vi "Test_tempo_realtime.vi"() -> ()   [LabVIEW 2017]
uses:
  <vilib>/Platform/TimedLoop/XDataNode/XDataNode.xnode
  <vilib>/Platform/TimedLoop/XDataNode/nitl_modes.ctl
  <vilib>/Platform/TimedLoop/XDataNode/XDNodeRunTimeDep.lvlib
  <vilib>/Platform/TimedLoop/XDataNode/wakeup.ctl
  <vilib>/Platform/TimedLoop/XDataNode/timing_clust.ctl
panel:
  out "Timer":u32 caption="Tick Count(mSec)"
  out "Tempo":bool
  in  "Timer":u32
  in  "Tempo":bool
  out "VI END":bool=TRUE
  out "Etat VI":enum16{""}(ring)
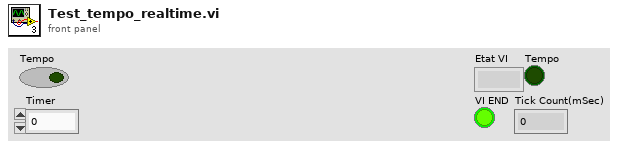
[diagram p1: front panel]
types:
  T1 = typedef "XDNodeRunTimeDep.lvlib/timing_clust.ctl" = cluster{"Expected End [f-1]":u64, "Actual End [f-1]":u64, "Finished Late? [f-1]":bool, "Expected End [i-1]":u64, "Actual End [i-1]":u64, "Finished Late? [i-1]":bool, "Expected Start [i]":u64, "Actual Start [i]":u64, "Expected Start [f]":u64, "Actual Start [f]":u64, "Source Name":string, "Structure Name":string, "Period":i64, "Deadline":i64, "Offset":i64, "Start":i64, "Priority":i32, "Timeout":i32, "Mode":T2, "Wakeup Reason":T3, "Error":errorcluster, "Source Type":string, "Secondary Source Type":string, "Global End Time":u64, "Global Start Time":u64, "Frame Duration":u64, "Iteration Duration":u64, "Assigned CPU":i32, "I/O Scan Engine Mode":u32}
  T2 = typedef "XDNodeRunTimeDep.lvlib/nitl_modes.ctl" = enum32{"No Change", "Process missed periods, maintain original phase", "Discard missed periods, maintain original phase", "Process missed periods, ignore original phase", "Discard missed periods, ignore original phase"}
  T3 = typedef "XDNodeRunTimeDep.lvlib/wakeup.ctl" = enum32{"Normal", "Aborted", "Asynchronous wakeup", "Timing source error", "Timed loop error", "Timeout"}
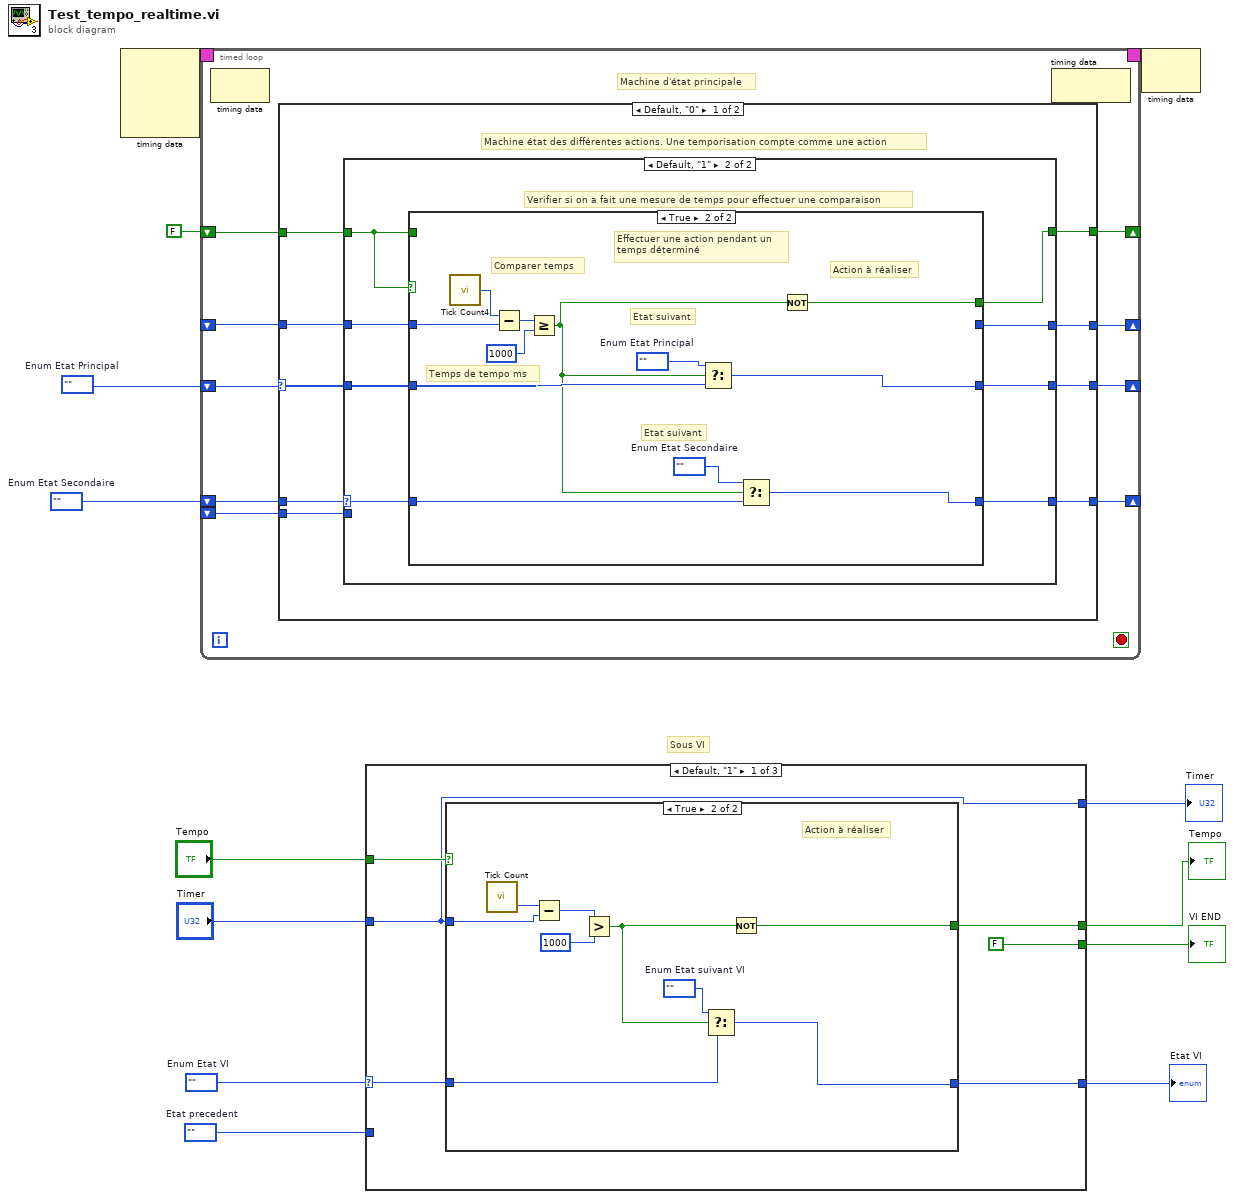
[diagram p0: block diagram]
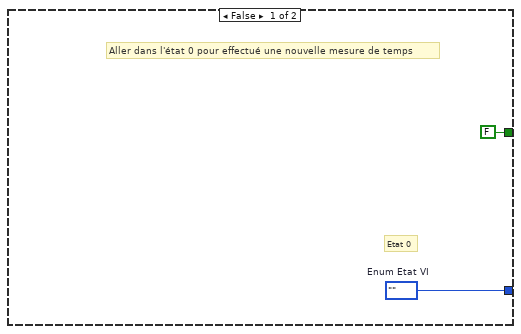
[diagram p2: hidden frame]
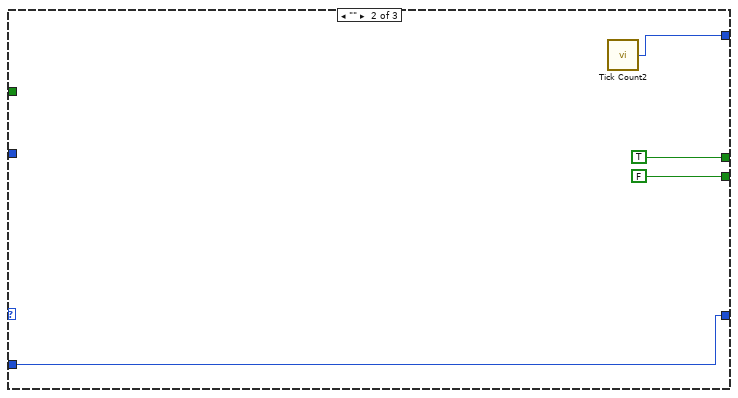
[diagram p3: hidden frame]
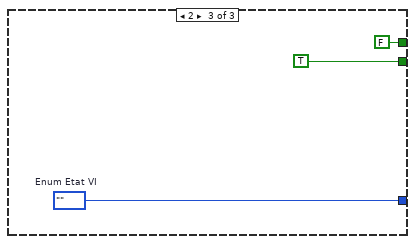
[diagram p4: hidden frame]
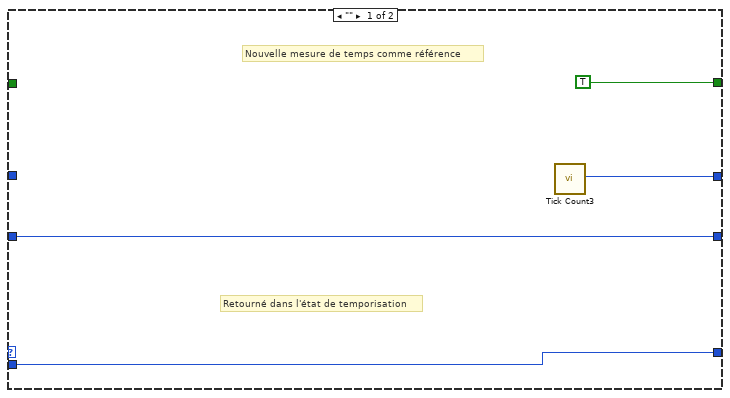
[diagram p5: hidden frame]
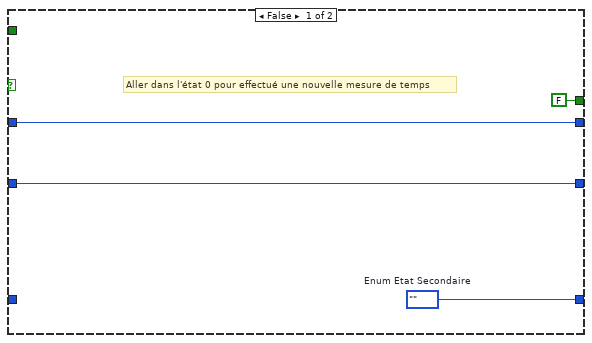
[diagram p6: hidden frame]
diagram:
  w2 = enum16{""}.""  # Etat precedent
  w1 = enum16{""}.""  # Enum Etat VI
  w10 = enum16{""}.""  # Enum Etat Secondaire
  w11 = enum16{""}.""  # Enum Etat Principal
  # "Sous VI"
  n1 = node-c288() -> (w13:T1)  [unwired: 4 in]
  n2 = timed-loop {
    timing: w13 -> [_]
    timing-out: [_] -> w12
    shift-right: [w16] -> _
    shift-left: w11 -> [w22]
    shift-right: [w18] -> _
    shift-left: w10 -> [w21]
    shift-right: [w20] -> _
    shift-left: _ -> [w19]
    shift-left: _ -> [w15]
    shift-right: [w17] -> _
    shift-left: FALSE -> [w14]
    stop <- _ stop-if-true
    # "Machine d'état principale"
    n3 = node-c288() -> ()  [unwired: 1 in, 1 out]
    n4 = case shown="Default, \"0\"" w22 {
      selector: w22 -> [w26 _]
      tunnel: w21 -> [w31 _]
      tunnel: [w30 _] -> w20
      tunnel: w19 -> [w29 _]
      tunnel: [w28 _] -> w18
      tunnel: [w27 _] -> w17
      tunnel: [w25 _] -> w16
      tunnel: w15 -> [w24 _]
      tunnel: w14 -> [w23 _]
      frame "", Default {
        # "Machine état des différentes actions. Une temporisation compte comme une action"
        n5 = case shown="Default, \"1\"" w31 {
          selector: w31 -> [_ w38]
          tunnel: [w35 w39] -> w30
          tunnel: w29 -> [_ w40]
          tunnel: [w32 w43] -> w28
          tunnel: [TRUE w36] -> w27
          tunnel: w26 -> [w33 w42]
          tunnel: [w33 w41] -> w25
          tunnel: w24 -> [w32 _]
          tunnel: w23 -> [_ w37]
          frame "" {
            # "Retourné dans l'état de temporisation"
            # "Nouvelle mesure de temps comme référence"
            n6 = call "Tick Count3"() -> ("Tick Count(mSec)"=w35:u32)
          }
          frame 1, Default {
            # "Verifier si on a fait une mesure de temps pour effectuer une comparaison"
            n7 = case shown="True" w37 {
              tunnel: [w47 w55] -> w43
              tunnel: w42 -> [w46 w52]
              tunnel: [w46 w51] -> w41
              tunnel: w40 -> [w45 w58]
              tunnel: [w45 _] -> w39
              tunnel: w38 -> [_ w54]
              tunnel: w37 -> [_ _]
              tunnel: [FALSE w49] -> w36
              frame False {
                w47 = enum16{""}.""  # Enum Etat Secondaire
                # "Aller dans l'état 0 pour effectué une nouvelle mesure de temps"
              }
              frame True {
                w48 = enum16{""}.""  # Enum Etat Principal
                w53 = enum16{""}.""  # Enum Etat Secondaire
                # "Temps de tempo ms"
                # "Effectuer une action pendant un\ntemps déterminé"
                # "Comparer temps"
                # "Etat suivant"
                # "Etat suivant"
                # "Action à réaliser"
                n8 = call "Tick Count4"() -> ("Tick Count(mSec)"=w59:u32)
                n9 = Subtract(x=w59, y=w58) -> (x-y=w57:u32)
                n10 = Greater Or Equal?(x=w57, y=u32 1000) -> (x >= y?=w50:bool)
                n11 = Select(t=w48, s=w50, f=w52) -> (s? t:f=w51:enum16{""})
                n12 = Select(t=w53, s=w50, f=w54) -> (s? t:f=w55:enum16{""})
                n13 = Not(x=w50) -> (.not. x?=w49:bool)
              }
            }
          }
        }
      }
      frame 1 {
      }
    }
    n14 = node-c288() -> ()  [unwired: 1 in, 1 out]
  }
  n15 = case shown="Default, \"1\"" w1 {
    selector: w1 -> [w65 _ _]
    tunnel: [w64 w79 w85] -> w8
    tunnel: [FALSE FALSE TRUE] -> w7
    tunnel: "Tempo" -> [w66 _ _]
    tunnel: "Timer" -> [w62 _ _]
    tunnel: [w63 TRUE FALSE] -> w4
    tunnel: [w62 w80 _] -> w3
    tunnel: w2 -> [_ w79 _]
    frame 1, Default {
      n16 = case shown="True" w66 {
        tunnel: w62 -> [_ w77]
        tunnel: w65 -> [_ w74]
        tunnel: [w69 w72] -> w64
        tunnel: [FALSE w70] -> w63
        frame False {
          w69 = enum16{""}.""  # Enum Etat VI
          # "Etat 0"
          # "Aller dans l'état 0 pour effectué une nouvelle mesure de temps"
        }
        frame True {
          w73 = enum16{""}.""  # Enum Etat suivant VI
          # "Action à réaliser"
          n17 = call "Tick Count"() -> ("Tick Count(mSec)"=w78:u32)
          n18 = Subtract(x=w78, y=w77) -> (x-y=w76:u32)
          n19 = Greater?(x=w76, y=u32 1000) -> (0:w71:bool)
          n20 = Select(t=w73, s=w71, f=w74) -> (s? t:f=w72:enum16{""})
          n21 = Not(x=w71) -> (.not. x?=w70:bool)
        }
      }
    }
    frame "" {
      n22 = call "Tick Count2"() -> ("Tick Count(mSec)"=w80:u32)
    }
    frame 2 {
      w85 = enum16{""}.""  # Enum Etat VI
    }
  }
  "Etat VI" <- w8
  "VI END" <- w7
  "Tempo" <- w4
  "Timer" <- w3
  n23 = node-c288(w12) -> ()  [unwired: 1 out]
